vi "Init.vi"(8 "error in (no error)":errorcluster, 9 "Config File Path":path=path "", 10 "Name":string, 11 "Base In":refnum<class "Base.lvclass">) -> (0 "error out":errorcluster, 3 "Base Out":refnum<class "Base.lvclass">)   [LabVIEW 2020, in "Base.lvclass"]
doc: "Initialize the class and creates necessary references. Anything initialized here is released in the Clear.vi method."
uses:
  Base.lvclass
  Base.lvclass/Base.ctl
  Private/SubVIs/Get Default Config Path.vi
  <vilib>/Utility/file.llb/Is Path and Not Empty.vi
  <vilib>/Utility/file.llb/Application Directory.vi
  <vilib>/Utility/error.llb/Error Cluster From Error Code.vi
  <vilib>/Utility/libraryn.llb/Check if File or Folder Exists.vi
  <vilib>/Utility/libraryn.llb/Create File and Containing Folders.vi
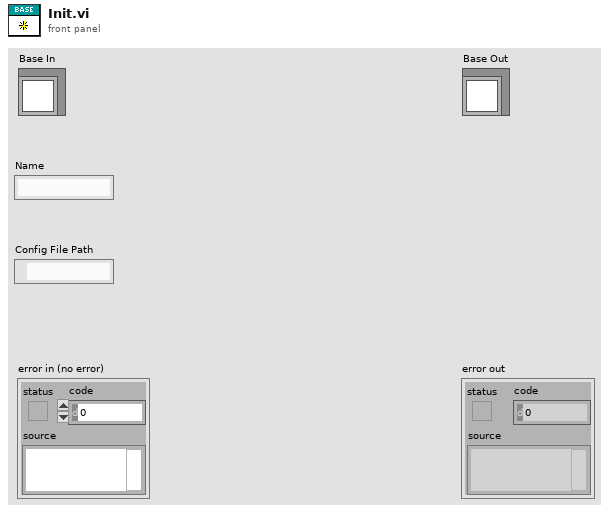
[diagram p1: front panel]
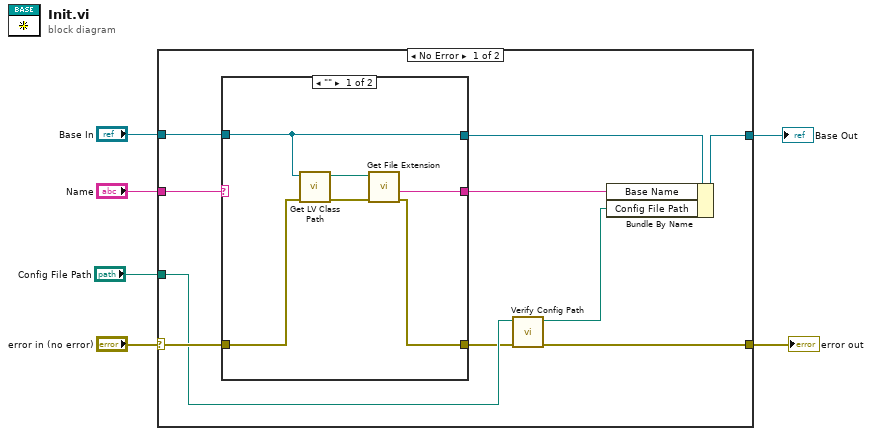
[diagram p0: block diagram]
diagram:
  n1 = case shown="No Error" "error in (no error)" {
    selector: "error in (no error)" -> [w12 w26]
    tunnel: [w16 w27] -> w6
    tunnel: "Base In" -> [w15 w27]
    tunnel: "Name" -> [w13 _]
    tunnel: "Config File Path" -> [w11 _]
    tunnel: [w8 w26] -> w1
    frame No Error {
      n2 = case shown="\"\"" w13 {
        selector: w13 -> [_ w23]
        tunnel: [w18 w23] -> w7
        tunnel: w15 -> [w17 w25]
        tunnel: w12 -> [w20 w24]
        tunnel: [w19 w24] -> w10
        tunnel: [w17 w25] -> w14
        frame "" {
          n3 = call <vilib>:"Get LV Class Path.vi"("error in (no error)"=w20, "object"=w17) -> ("error out"=w21:errorcluster, "class path"=w22:path)  [unwired: 8 in]
          n4 = call <vilib>:"Get File Extension.vi"("error in (no error)"=w21, "file"=w22) -> ("error out"=w19:errorcluster, "filename without extension"=w18:string)  [unwired: 5 in, 3 out]
        }
        frame Default {
          # "The name should be unique for each process in an application context. Multiple contexts may have processes with the same names without conflicts as the name is qualified within the context."
        }
      }
      n5 = call "Verify Config Path.vi"("error in (no error)"=w10, "Config File Path"=w11) -> ("error out"=w8:errorcluster, "dup path"=w9:path)  [unwired: 8 in]
      n6 = Bundle By Name(cluster=w14, "Base Name"=w7, "Config File Path"=w9) -> (w16:refnum<class "Base.lvclass">)
    }
    frame Error {
    }
  }
  "error out" <- w1
  "Base Out" <- w6
